vi "Sodium Boiler Model.vi"(5 "Heated Coolant Input (mB/t)":i64, 11 "Build Specifications":T1={"Length (m)"=5, "Width (m)"=5, "Superheating Elements"=3, "Water Cavity Height (m)"=0, "Steam Cavity Height (m)"=0} {"Superheating Elements" min=1 max=2 step=1; "Width (m)" min=5 max=17 step=2; "Length (m)" min=5 max=17 step=2}) -> (4 "Computed Build Properties":T2={"Water Tank (mB)"=0, "Steam Tank (mB)"=0, "Heated Coolant Tank (mB)"=0, "Coolant Tank (mB)"=0, "Maximum Boil Rate (mB/t)"=4, "Height (m)"=4, "Volume (m³)"=0, "Heat Capacity (J/K)"=0.0, "Pressure Dispersers"=4} {"Pressure Dispersers" min=4 max=18 step=1; "Height (m)" min=4 max=18 step=1; "Maximum Boil Rate (mB/t)" min=4 max=18 step=1})   [LabVIEW 2026]
uses:
  Boiler Build Properties.ctl
  Boiler Build Specifications.ctl
panel:
  out "Steam Tubes Required":u32=4 min=4 max=18 step=1
  out "Status":bool
  out "Water Demand (mB/t)":i64
  out "Boil Rate (mB/t)":dbl(slide) scale=0.0..960000.0 scale format="%#_6f"
  out "Sodium Loops Required":u32=4 min=4 max=18 step=1
  out "Water Pipes Required":u32=4 min=4 max=18 step=1
  out "Steam Output (mB/t)":i64
  out "Coolant Output (mB/t)":i64
  # "Thermoelectric Boiler Properties"
  # "Note: The boiler's heated coolant tank size must be about twice the size of the\nreactor's coolant tank, with as much coolant buffered in the coolant return tube\nand as much water as the water tank's capacity buffered in the water return tubes."
  # "Thermoelectric Boiler Operation"
  # "+1 for heating elements"
  # "+1 for dispersers"
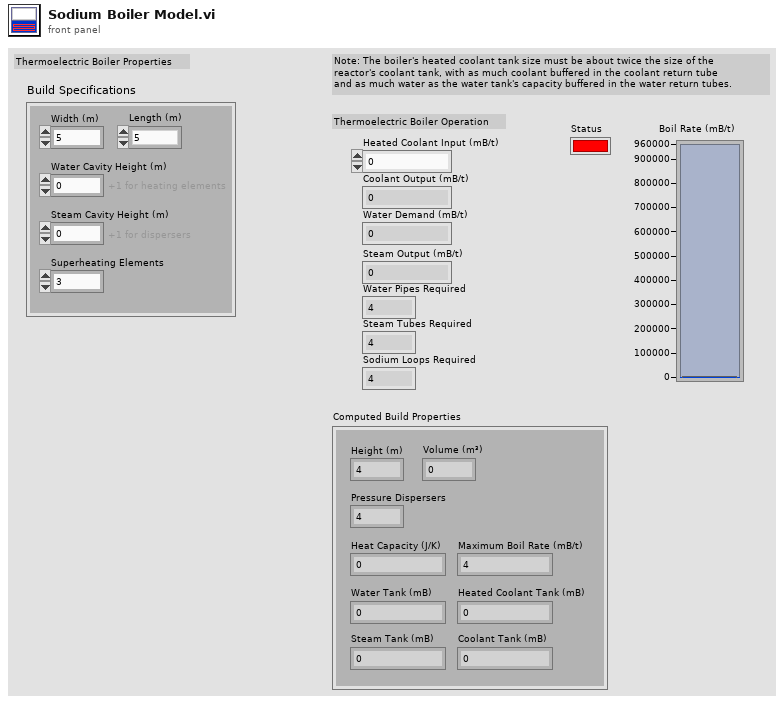
[diagram p1: front panel]
types:
  T1 = typedef "Boiler Build Specifications.ctl" = cluster{"Length (m)":i32, "Width (m)":i32, "Superheating Elements":i32, "Water Cavity Height (m)":i32, "Steam Cavity Height (m)":i32}
  T2 = typedef "Boiler Build Properties.ctl" = cluster{"Water Tank (mB)":i32, "Steam Tank (mB)":i32, "Heated Coolant Tank (mB)":i64, "Coolant Tank (mB)":i64, "Maximum Boil Rate (mB/t)":i32, "Height (m)":i32, "Volume (m³)":i32, "Heat Capacity (J/K)":dbl, "Pressure Dispersers":i32}
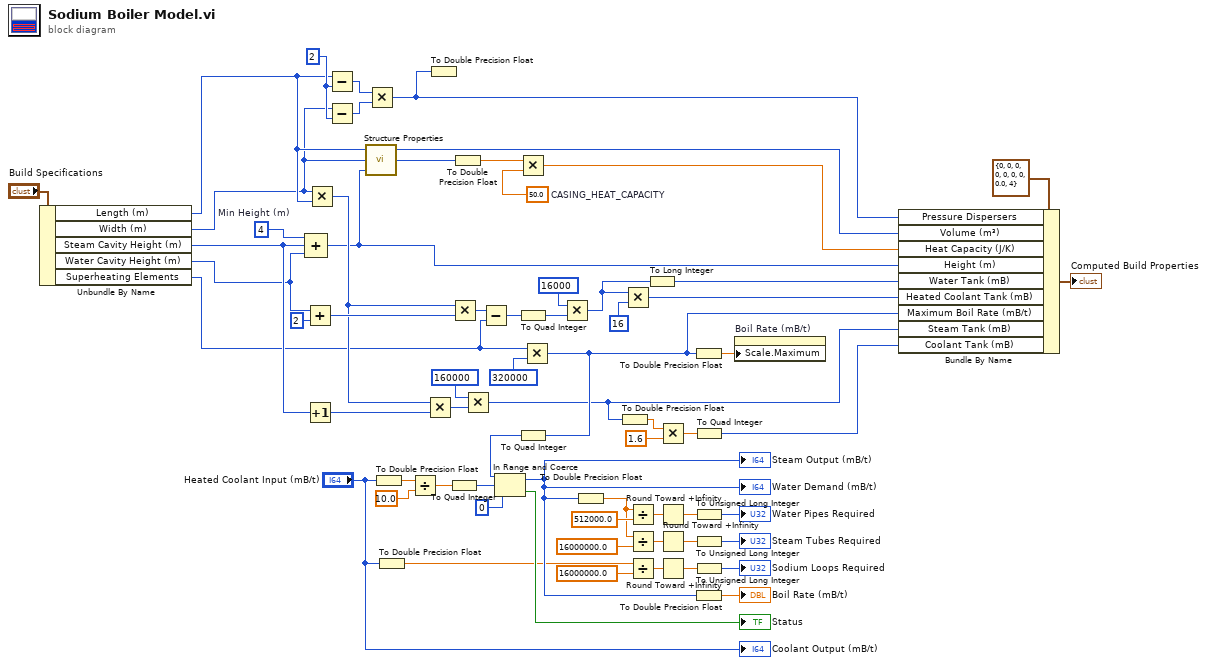
[diagram p0: block diagram]
diagram:
  w12 = 50.0  # CASING_HEAT_CAPACITY
  w60 = 2 ("y")
  w65 = 4  # Min Height (m)
  n1 = Unbundle By Name("Build Specifications") -> ("Length (m)"=w5:i32, "Width (m)"=w4:i32, "Steam Cavity Height (m)"=w3:i32, "Water Cavity Height (m)"=w2:i32, "Superheating Elements"=w1:i32)
  n2 = Compound Arithmetic op=ADD(w65, w3, w2) -> (w14:i32)
  n3 = Add(x=w2, y=2) -> (x+y=w51:i32)
  n4 = Increment(x=w3) -> (x+1=w49:i32)
  n5 = Multiply(x=w4, y=w5) -> (x*y=w50:i32)
  n6 = Subtract(x=w5, y=w60) -> (x-y=w59:i32)
  n7 = Subtract(x=w4, y=w60) -> (x-y=w58:i32)
  n8 = call "Structure Properties.vi"("Length"=w5, "Width"=w4, "Height"=w14) -> ("Volume"=w8:i32, "Casing"=w10:i32)  [unwired: 2 in, 3 out]
  n9 = Multiply(x=w59, y=w58) -> (x*y=w9:i32)
  n10 = To Double Precision Float(number="Heated Coolant Input (mB/t)") -> (double precision float=w37:dbl)
  n11 = To Double Precision Float(number="Heated Coolant Input (mB/t)") -> (double precision float=w29:dbl)
  n12 = Divide(x=w37, y=10.0) -> (x/y=w38:dbl)
  n13 = Multiply(x=w50, y=w49) -> (x*y=w54:i32)
  n14 = To Double Precision Float(number=w9) -> ()  [unwired: 1 out]
  n15 = To Quad Integer(1:w38) -> (0:w35:i64)
  n16 = Multiply(x=w50, y=w51) -> (x*y=w63:i32)
  n17 = To Double Precision Float(number=w10) -> (double precision float=w11:dbl)
  n18 = Multiply(x=160000 ("y"), y=w54) -> (x*y=w15:i32)
  n19 = Subtract(x=w63, y=w1) -> (x-y=w61:i32)
  n20 = Multiply(x=w11, y=w12) -> (x*y=w7:dbl)
  n21 = To Quad Integer(1:w61) -> (0:w22:i64)
  n22 = Multiply(x=w1, y=320000) -> (x*y=w16:i32)
  n23 = To Quad Integer(1:w16) -> (0:w21:i64)
  n24 = In Range and Coerce(upper limit=w21, x=w35, lower limit=i64 0) -> (coerced(x)=w31:i64, In Range?=→"Status":bool)
  "Steam Output (mB/t)" <- w31
  "Water Demand (mB/t)" <- w31
  n25 = Multiply(x=i64 16000 ("y"), y=w22) -> (x*y=w57:i64)
  n26 = To Double Precision Float(number=w31) -> (double precision float=w23:dbl)
  n27 = To Double Precision Float(number=w15) -> (double precision float=w33:dbl)
  n28 = Multiply(x=w57, y=i64 16) -> (x*y=w17:i64)
  n29 = Divide(x=w23, y=512000.0) -> (x/y=w45:dbl)
  n30 = Divide(x=w23, y=16000000.0) -> (x/y=w25:dbl)
  n31 = Divide(x=w29, y=16000000.0) -> (x/y=w44:dbl)
  n32 = To Long Integer(number=w57) -> (32bit integer=w19:i32)
  n33 = Multiply(x=w33, y=1.6) -> (x*y=w52:dbl)
  n34 = Round Toward +Infinity(x=w45) -> (ceil(x): smallest int >= x=w43:dbl)
  n35 = Round Toward +Infinity(x=w25) -> (ceil(x): smallest int >= x=w26:dbl)
  n36 = Round Toward +Infinity(x=w44) -> (ceil(x): smallest int >= x=w42:dbl)
  n37 = To Double Precision Float(number=w16) -> (double precision float=w32:dbl)
  n38 = To Quad Integer(1:w52) -> (0:w13:i64)
  n39 = To Unsigned Long Integer(number=w43) -> (unsigned 32bit integer=→"Water Pipes Required":u32)
  n40 = To Unsigned Long Integer(number=w26) -> (unsigned 32bit integer=→"Steam Tubes Required":u32)
  n41 = To Unsigned Long Integer(number=w42) -> (unsigned 32bit integer=→"Sodium Loops Required":u32)
  n42 = To Double Precision Float(number=w31) -> (double precision float=→"Boil Rate (mB/t)":dbl)
  n43 = property on="Boil Rate (mB/t)" class="Slide (strict)"("Scale.Maximum"=w32) -> ()  [unwired: 2 in, 2 out]
  n44 = Bundle By Name(cluster=T2 {"Water Tank (mB)"=0, "Steam Tank (mB)"=0, "Heated Coolant Tank (mB)"=0, "Coolant Tank (mB)"=0, "Maximum Boil Rate (mB/t)"=0, "Height (m)"=0, "Volume (m³)"=0, "Heat Capacity (J/K)"=0.0, "Pressure Dispersers"=4} ("Boiler Build Properties"), "Pressure Dispersers"=w9, "Volume (m³)"=w8, "Heat Capacity (J/K)"=w7, "Height (m)"=w14, "Water Tank (mB)"=w19, "Heated Coolant Tank (mB)"=w17, "Maximum Boil Rate (mB/t)"=w16, "Steam Tank (mB)"=w15, "Coolant Tank (mB)"=w13) -> (→"Computed Build Properties":T2)
  "Coolant Output (mB/t)" <- "Heated Coolant Input (mB/t)"
